vi "Read remotePort.vi"(8 "error in (no error)":errorcluster, 11 "ZM-CP-UDP-sender in":refnum<class "ZM-CP-UDP-sender.lvclass">) -> (0 "error out":errorcluster, 2 "remotePort":u16=61557, 3 "ZM-CP-UDP-sender out":refnum<class "ZM-CP-UDP-sender.lvclass">)   [LabVIEW 2020, in "ZM-CP-UDP-udp_transport.lvlib" / "ZM-CP-UDP-sender.lvclass"]
doc: "Reads one field of this class's private data. Generated by lvai_create_accessors from the class private data control."
uses:
  ZM-CP-UDP-sender.lvclass
  ZM-CP-UDP-sender.lvclass/ZM-CP-UDP-sender.ctl
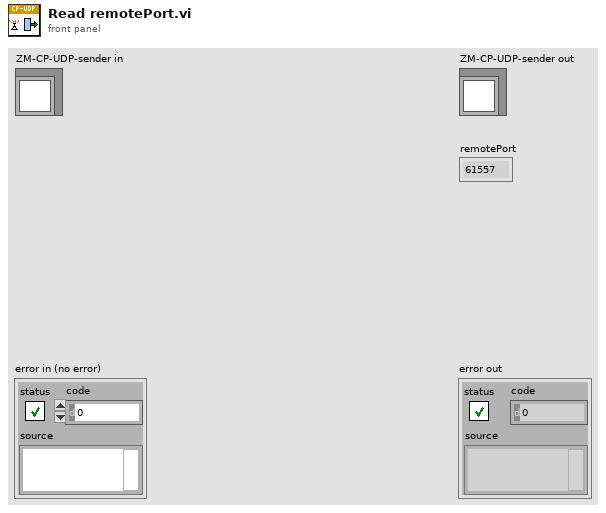
[diagram p1: front panel]
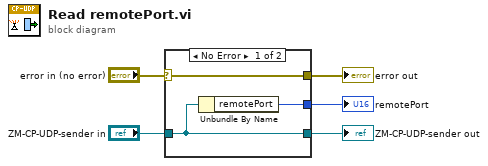
[diagram p0: block diagram]
diagram:
  n1 = case shown="No Error" "error in (no error)" {
    selector: "error in (no error)" -> [w8 w9]
    tunnel: [w8 w9] -> w4
    tunnel: [w7 w10] -> w2
    tunnel: "ZM-CP-UDP-sender in" -> [w7 w10]
    tunnel: [w6 _] -> w1
    frame No Error {
      n2 = Unbundle By Name(w7) -> ("remotePort"=w6:u16)
    }
    frame Error {
    }
  }
  "error out" <- w4
  "ZM-CP-UDP-sender out" <- w2
  "remotePort" <- w1
